vi "Get array of DBL.vi"(8 "error in (no error)":errorcluster, 10 "Name":string, 11 "json class in":refnum<class "json class.lvclass">) -> (0 "error out":errorcluster, 2 "DBL Array":dbl[](array[numeric]), 3 "json class out":refnum<class "json class.lvclass">)   [LabVIEW 2021, in "Config Library.lvlib" / "json class.lvclass"]
uses:
  json class.lvclass
  json class.lvclass/json class.ctl
  <vilib>/addons/JSON API/JSON Value/JSON Value.lvclass
  <vilib>/addons/JSON API/JSON Array/JSON Array.lvclass
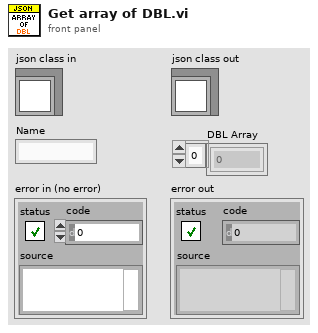
[diagram p1: front panel]
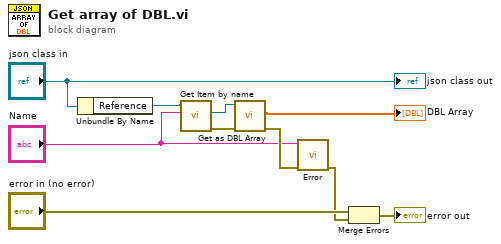
[diagram p0: block diagram]
diagram:
  n1 = Unbundle By Name("json class in") -> ("Reference"=w4:refnum<class "JSON Value.lvclass">)
  n2 = call-dynamic "Get Item by name.vi"("name"="Name", "JSON Value In"=w4) -> ("error out"=w2:errorcluster, "Value"=w3:refnum<class "JSON Value.lvclass">)  [unwired: 6 in, 2 out]
  n3 = call <vilib>:"Get as DBL Array.vi"("error in (no error)"=w2, "JSON Array in"=w3) -> ("error out"=w6:errorcluster, "Array of numbers"=→"DBL Array":dbl[])  [unwired: 7 in, 1 out]
  n4 = call "Error.vi"("error in (no error)"=w6, "Name"="Name") -> ("error out"=w5:errorcluster)  [unwired: 9 in]
  n5 = Merge Errors("error in (no error)", w5) -> (→"error out":errorcluster)
  "json class out" <- "json class in"
